vi "filter tags by owner.vi"(9 "exclude? (default: include)":bool, 10 "owner":string, 11 "engine configuration in":refnum<class "engine configuration.lvclass">) -> (2 "tag list":refnum<class "tag descriptor.lvclass">[](array[class]), 3 "engine configuration out":refnum<class "engine configuration.lvclass">)   [LabVIEW 2014, in "engine configuration.lvclass"]
doc: "Returns a list of tags that are owned by the identifier specifed in the 'owner' input."
uses:
  engine configuration.lvclass
  <vilib>/NI/Tag Bus/tag/tag descriptor.lvclass
  engine configuration.lvclass/engine configuration.ctl
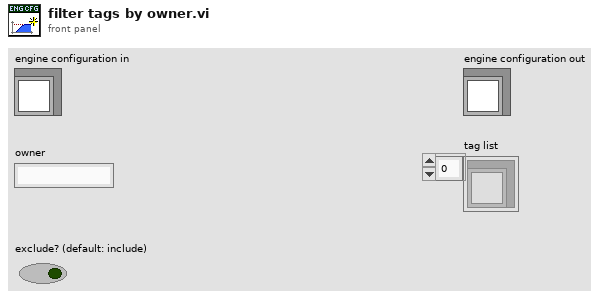
[diagram p1: front panel]
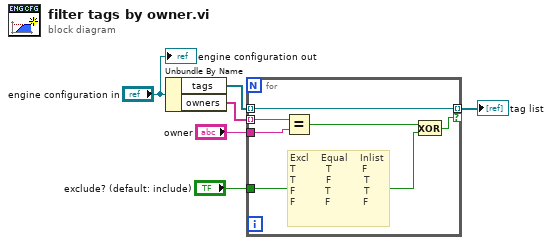
[diagram p0: block diagram]
diagram:
  n1 = Unbundle By Name("engine configuration in") -> ("tags"=w1:refnum<class "tag descriptor.lvclass">[], "owners"=w2:string[])
  n2 = for {
    tunnel: [w7] -> w5 mode=indexing if=w9
    tunnel: "exclude? (default: include)" -> [w10]
    tunnel: "owner" -> [w12]
    tunnel: w2 -> [w8] mode=indexing
    tunnel: w1 -> [w7] mode=indexing
    # "Excl    Equal    Inlist\nT          T          F \nT          F           T\nF          T           T\nF          F           F"
    n3 = Equal?(x=w8, y=w12) -> (x = y?=w11:bool)
    n4 = Exclusive Or(1:w10, 2:w11) -> (0:w9:bool)
  }
  "tag list" <- w5
  "engine configuration out" <- "engine configuration in"
